vi "SA set TDF ON.vi"(8 "error in (no error)":errorcluster caption="에러 입력(에러 없음)", 10 "TDF File Name":string, 11 "Instrument Manager 입력":refnum<class "Instrument Manager.lvclass">) -> (0 "error out":errorcluster caption="에러 출력", 3 "Instrument Manager 출력":refnum<class "Instrument Manager.lvclass">)   [LabVIEW 2023, in "Instrument Manager.lvclass"]
uses:
  Instrument Manager.lvclass
  Instrument Manager.lvclass/Instrument Manager.ctl
  84f9a906-5752-46b4-8268-c74757d55e67.vi
  d5135b29-b1b1-43ef-a158-dd08169a51d8.vi
  Module/Spectrum Analyzer/Interface_Spectrum/Interface_Spectrum.lvclass
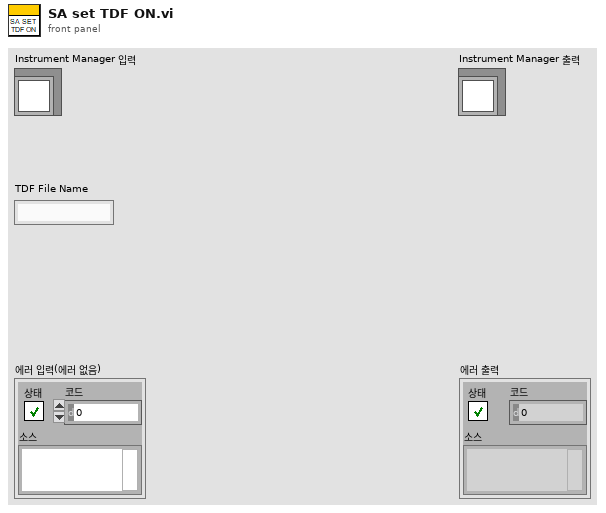
[diagram p1: front panel]
types:
  T1 = cluster{"Anritsu Call Box":refnum<class "Anritsu Call Box.lvclass">, "Spectrum Analyzer":refnum<class "Interface_Spectrum.lvclass">, "RF Switch Box":refnum<class "RF Filter Box.lvclass">, "Turn Table":refnum<class "Interface - Turn Table.lvclass">, "Mast":refnum<class "Interface - Mast.lvclass">, "3D Controller":refnum<class "Interface_3D Controller.lvclass">}
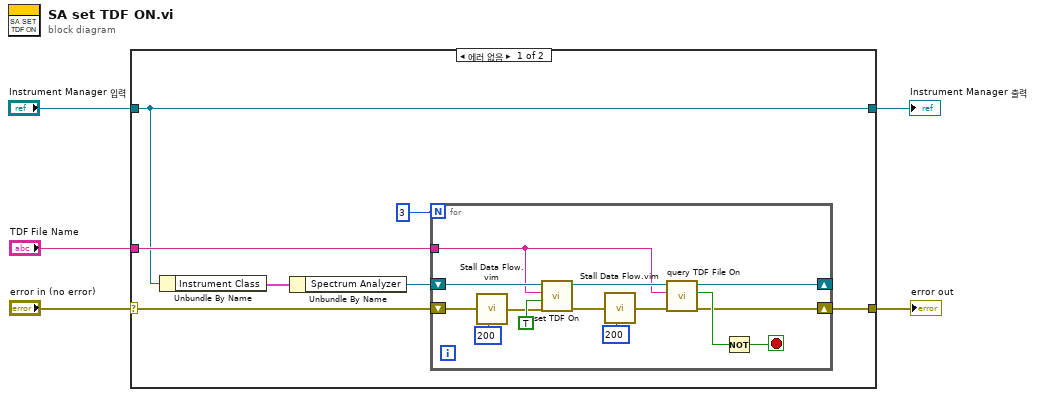
[diagram p0: block diagram]
diagram:
  n1 = case shown="에러 없음" "error in (no error)" {
    selector: "error in (no error)" -> [w12 w28]
    tunnel: [w11 w28] -> w4
    tunnel: [w9 w27] -> w2
    tunnel: "Instrument Manager 입력" -> [w9 w27]
    tunnel: "TDF File Name" -> [w10 _]
    frame No Error {
      n2 = Unbundle By Name(w9) -> ("Instrument Class"=w8:T1)
      n3 = Unbundle By Name(w8) -> ("Spectrum Analyzer"=w7:refnum<class "Interface_Spectrum.lvclass">)
      n4 = for {
        N: 3 -> [_]
        shift-right: [w20] -> w11
        shift-left: w12 -> [w14]
        shift-right: [w19] -> _
        shift-left: w7 -> [w26]
        tunnel: w10 -> [w23]
        stop <- w21 stop-if-true
        n5 = call "Stall Data Flow.vim"("value in"=w14, "milliseconds to wait"=u32 200) -> ("value out"=w13:errorcluster)  [unwired: 1 out]
        n6 = call-dynamic "set TDF On.vi"("error in (no error)"=w13, "On?"=TRUE, "File Name"=w23, "Interface_Spectrum 입력"=w26) -> ("error out"=w18:errorcluster, "Interface_Spectrum 출력"=w25:refnum<class "Interface_Spectrum.lvclass">)  [unwired: 6 in]
        n7 = call "Stall Data Flow.vim"("value in"=w18, "milliseconds to wait"=u32 200) -> ("value out"=w17:errorcluster)  [unwired: 1 out]
        n8 = call-dynamic "query TDF File On.vi"("error in (no error)"=w17, "File Name"=w23, "Interface_Spectrum 입력"=w25) -> ("error out"=w20:errorcluster, "On?"=w22:bool, "Interface_Spectrum 출력"=w19:refnum<class "Interface_Spectrum.lvclass">)  [unwired: 6 in]
        n9 = Not(x=w22) -> (.not. x?=w21:bool)
      }
    }
    frame Error {
    }
  }
  "error out" <- w4
  "Instrument Manager 출력" <- w2
